vi "SetDutyCycle.vi"(8 "error in (no error)":errorcluster, 10 "Duty Cycles":sgl[](array[numeric]), 11 "M5Stack I2C 8Ch Servo in":refnum<class "M5Stack I2C 8Ch Servo.lvclass">) -> (0 "error out":errorcluster, 3 "M5Stack I2C 8Ch Servo out":refnum<class "M5Stack I2C 8Ch Servo.lvclass">)   [LabVIEW 2020, in "CTI-Peripheral.lvlib" / "M5Stack I2C 8Ch Servo.lvclass"]
uses:
  M5Stack I2C 8Ch Servo.lvclass
  M5Stack I2C 8Ch Servo.lvclass/M5Stack I2C 8Ch Servo.ctl
  Private/registers.ctl
  CTI/I2C Connection/I2C Connection.lvclass/I2C Connection.ctl
  CTI/Session/I2C Write Data.vi
  CTI/I2C Connection/I2C Connection.lvclass
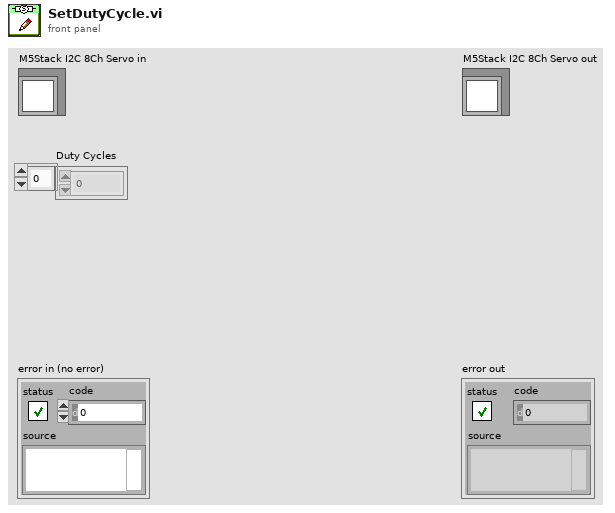
[diagram p1: front panel]
types:
  T1 = typedef "CTI-Peripheral.lvlib/M5Stack I2C 8Ch Servo.lvclass/registers.ctl" = u8
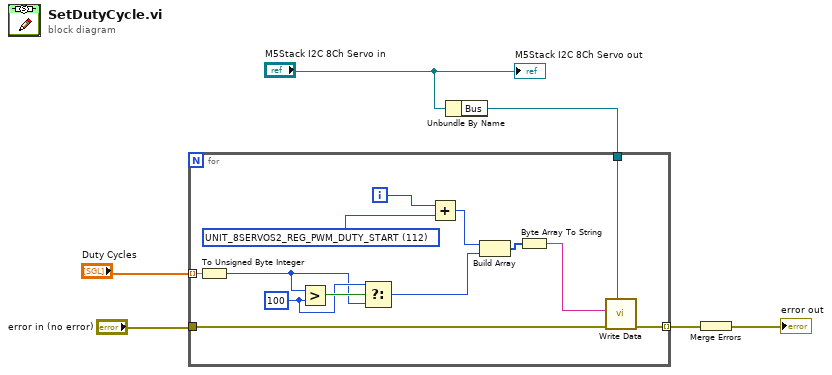
[diagram p0: block diagram]
diagram:
  n1 = Unbundle By Name("M5Stack I2C 8Ch Servo in") -> ("Bus"=w4:refnum<class "I2C Connection.lvclass">)
  n2 = for {
    tunnel: w4 -> [w14]
    tunnel: "Duty Cycles" -> [w11] mode=indexing
    tunnel: "error in (no error)" -> [w13]
    tunnel: [w16] -> w6 mode=indexing
    i -> [w12]
    w9 = u8 100 ("y")
    w17 = T1 112 items=["UNIT_8SERVOS2_REG_MODE_START"=0, "UNIT_8SERVOS2_REG_INPUT_PULL_START"=16, "UNIT_8SERVOS2_REG_INPUT_STATUS_START"=32, "UNIT_8SERVOS2_REG_OUTPUT_STATUS_START"=48, "UNIT_8SERVOS2_REG_ADC_START"=64, "UNIT_8SERVOS2_REG_SERVO_START"=80, "UNIT_8SERVOS2_REG_RGB_CONF_START"=96, "UNIT_8SERVOS2_REG_PWM_DUTY_START"=112, "UNIT_8SERVOS2_REG_RGB_BUFFER_START"=128, "UNIT_8SERVOS2_REG_TIM_FREQ_START"=208, "UNIT_8SERVOS2_REG_UID_START"=224, "UNIT_8SERVOS2_REG_UID_END"=235, "UNIT_8SERVOS2_REG_SYS_ANALOG_START"=240, "UNIT_8SERVOS2_REG_ADDR_OFFSET"=248, "UNIT_8SERVOS2_REG_I2C_ADDR_REFRESH"=252, "UNIT_8SERVOS2_REG_VERSION"=254, "UNIT_8SERVOS2_REG_I2C_ADDR"=255] ("Registers")
    n3 = To Unsigned Byte Integer(number=w11) -> (unsigned 8bit integer=w8:u8)
    n4 = Greater?(x=w8, y=w9) -> (0:w10:bool)
    n5 = Select(t=w9, s=w10, f=w8) -> (s? t:f=w7:u8)
    n6 = Add(x=w12, y=w17) -> (x+y=w18:i32)
    n7 = Build Array(w18, w7) -> (w19:i32[])
    n8 = Byte Array To String(unsigned byte array=w19) -> (string=w15:string)
    n9 = call "Write Data.vi"("I2C Connection"=w14, "error in (no error)"=w13, "Data"=w15) -> ("error out"=w16:errorcluster)  [unwired: 8 in]
  }
  n10 = Merge Errors(w6) -> (→"error out":errorcluster)
  "M5Stack I2C 8Ch Servo out" <- "M5Stack I2C 8Ch Servo in"
